vi "SetContextMenu.vi"(8 "error in (no error)":errorcluster, 11 "Gviewer in":refnum<class "Gviewer.lvclass">) -> (0 "error out":errorcluster, 3 "Gviewer out":refnum<class "Gviewer.lvclass">)   [LabVIEW 2020, in "Sgraph_lib_V1.lvlib" / "Gviewer.lvclass"]
doc: "Andre Koelewijn, 5 jan 2021\n\nSet or refresh the Contect (right mouse button) context menu structure"
uses:
  Gviewer.lvclass
  Gviewer.lvclass/Gviewer.ctl
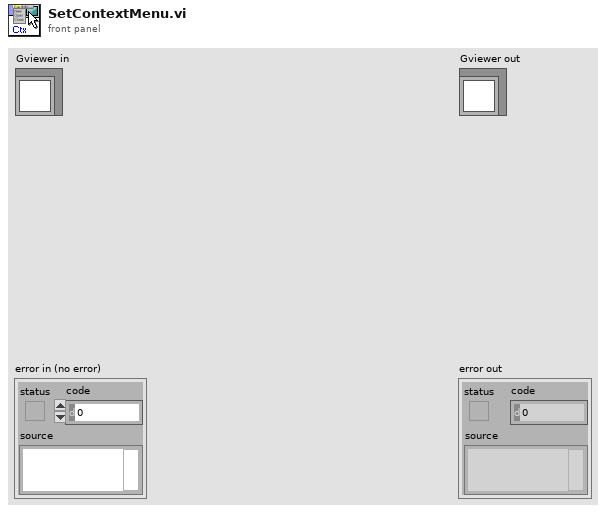
[diagram p1: front panel]
types:
  T1 = typedef "MenuItem.ctl" = cluster{"name":string, "tag":string, "checked":bool, "enabled":bool}
  T2 = typedef "MenuStructure.ctl" = cluster{"After_tag":string, "MenuItems":T1[]}[]
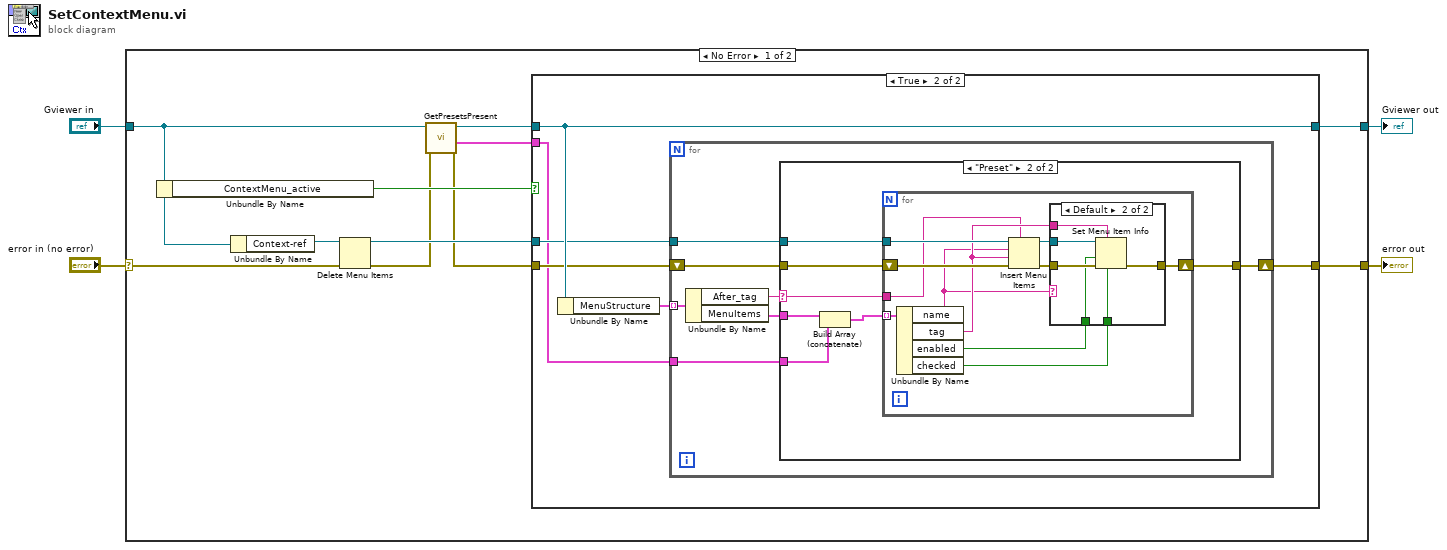
[diagram p0: block diagram]
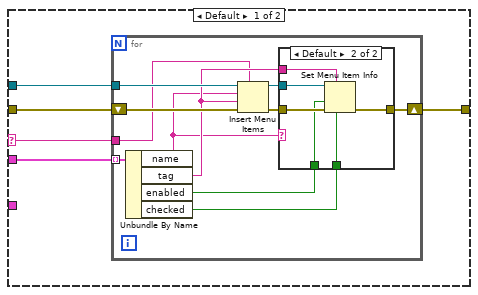
[diagram p3: hidden frame]
diagram:
  n1 = case shown="No Error" "error in (no error)" {
    selector: "error in (no error)" -> [w11 w80]
    tunnel: [w14 w80] -> w3
    tunnel: [w15 w79] -> w1
    tunnel: "Gviewer in" -> [w8 w79]
    frame No Error {
      n2 = Unbundle By Name(w8) -> ("ContextMenu_active"=w13:bool)
      n3 = Unbundle By Name(w8) -> ("Context-ref"=w12:refnum<k9>)
      n4 = Delete Menu Items(6:w11, 9:w12) -> (0:w7:errorcluster, 3:w10:refnum<k9>)  [unwired: 2 in]
      n5 = call "GetPresetsPresent.vi"("error in (no error)"=w7, "Gviewer in"=w8) -> ("error out"=w6:errorcluster, "PresentsInMenu"=w5:T1[], "Gviewer out"=w9:refnum<class "Gviewer.lvclass">)  [unwired: 7 in]
      n6 = case shown="True" w13 {
        tunnel: w9 -> [w17 w23]
        tunnel: [w17 w23] -> w15
        tunnel: [w16 w21] -> w14
        tunnel: w6 -> [w16 w19]
        tunnel: w10 -> [_ w20]
        tunnel: w5 -> [_ w18]
        frame False {
        }
        frame True {
          n7 = Unbundle By Name(w23) -> ("MenuStructure"=w22:T2)
          n8 = for {
            tunnel: w22 -> [w30] mode=indexing
            shift-right: [w26] -> w21
            shift-left: w19 -> [w27]
            tunnel: w20 -> [w25]
            tunnel: w18 -> [w24]
            n9 = Unbundle By Name(w30) -> ("After_tag"=w28:string, "MenuItems"=w29:T1[])
            n10 = case shown="\"Preset\"" w28 {
              selector: w28 -> [w34 w60]
              tunnel: w29 -> [w35 w55]
              tunnel: w27 -> [w33 w59]
              tunnel: [w32 w58] -> w26
              tunnel: w25 -> [w31 w57]
              tunnel: w24 -> [_ w54]
              frame Default {
                n11 = for {
                  tunnel: w35 -> [w43] mode=indexing
                  tunnel: w34 -> [w37]
                  shift-right: [w44] -> w32
                  shift-left: w33 -> [w46]
                  tunnel: w31 -> [w42]
                  n12 = Unbundle By Name(w43) -> ("name"=w36:string, "tag"=w38:string, "enabled"=w39:bool, "checked"=w40:bool)
                  n13 = Insert Menu Items(5:w37, 6:w46, 7:w38, 8:w36, 9:w42) -> (0:w45:errorcluster, 3:w41:refnum<k9>)  [unwired: 1 in, 1 out]
                  n14 = case shown="Default" w36 {
                    tunnel: w45 -> [w47 w53]
                    tunnel: [w47 w52] -> w44
                    tunnel: w41 -> [_ w51]
                    tunnel: w40 -> [_ w50]
                    tunnel: w39 -> [_ w49]
                    tunnel: w38 -> [_ w48]
                    frame "app_separator" {
                    }
                    frame Default {
                      n15 = Set Menu Item Info(6:w50, 7:w48, 8:w53, 9:w49, 11:w51) -> (0:w52:errorcluster)  [unwired: 2 in, 1 out]
                    }
                  }
                }
              }
              frame "Preset" {
                n16 = Build Array (concatenate)(w55, w54) -> (w56:T1[])
                n17 = for {
                  tunnel: w56 -> [w68] mode=indexing
                  tunnel: w60 -> [w62]
                  shift-right: [w69] -> w58
                  shift-left: w59 -> [w71]
                  tunnel: w57 -> [w67]
                  n18 = Unbundle By Name(w68) -> ("name"=w61:string, "tag"=w63:string, "enabled"=w64:bool, "checked"=w65:bool)
                  n19 = Insert Menu Items(5:w62, 6:w71, 7:w63, 8:w61, 9:w67) -> (0:w70:errorcluster, 3:w66:refnum<k9>)  [unwired: 1 in, 1 out]
                  n20 = case shown="Default" w61 {
                    tunnel: w70 -> [w72 w78]
                    tunnel: [w72 w77] -> w69
                    tunnel: w66 -> [_ w76]
                    tunnel: w65 -> [_ w75]
                    tunnel: w64 -> [_ w74]
                    tunnel: w63 -> [_ w73]
                    frame "app_separator" {
                    }
                    frame Default {
                      n21 = Set Menu Item Info(6:w75, 7:w73, 8:w78, 9:w74, 11:w76) -> (0:w77:errorcluster)  [unwired: 2 in, 1 out]
                    }
                  }
                }
              }
            }
          }
        }
      }
    }
    frame Error {
    }
  }
  "error out" <- w3
  "Gviewer out" <- w1
